vi "[ce] LM Fit - XX.vi"(5 "Standard Deviation ^2":dbl[](array[numeric]) format="%.2f", 6 "error in":errorcluster, 8 "Y":dbl[](array[numeric]) format="%.2f", 9 "coefficient values":dbl[](array[numeric]) format="%.2f") -> (0 "error out":errorcluster, 1 "calc formula result":dbl[](array[numeric]) format="%.2f", 3 "chiSqr":dbl format="%.2f")   [LabVIEW 2021]
doc: "::: CalcExpress Toolkit :::\nCopyright (c) 2000-2026 Konstantin Shifershteyn. All rights reserved."
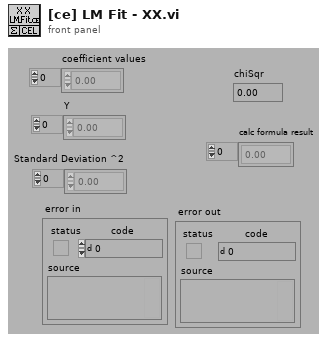
[diagram p1: front panel]
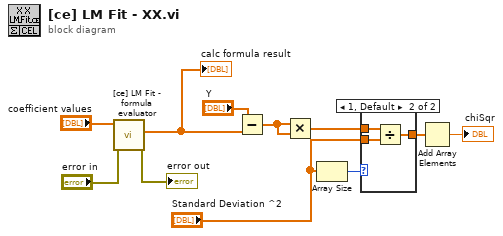
[diagram p0: block diagram]
diagram:
  n1 = call "[ce] LM Fit - formula evaluator.vi"("error in"="error in", "coef values"="coefficient values") -> ("error out"=→"error out":errorcluster, "calc result"=w4:dbl[])  [unwired: 7 in, 1 out]
  "calc formula result" <- w4
  n2 = Subtract(x="Y", y=w4) -> (x-y=w10:dbl[])
  n3 = Multiply(x=w10, y=w10) -> (x*y=w9:dbl[])
  n4 = Array Size(array="Standard Deviation ^2") -> (size(s)=w2:i32)
  n5 = case shown="1, Default" w2 {
    tunnel: w9 -> [w12 w15]
    tunnel: [w12 w14] -> w8
    tunnel: "Standard Deviation ^2" -> [_ w13]
    frame 0 {
    }
    frame 1, Default {
      n6 = Divide(x=w15, y=w13) -> (x/y=w14:dbl[])
    }
  }
  n7 = Add Array Elements(numeric array=w8) -> (sum=→"chiSqr":dbl)
